vi "Run.vi"(8 "error in (no error)":errorcluster, 11 "LINX in":refnum<class "LINX.lvclass">) -> (0 "error out":errorcluster, 3 "LINX out":refnum<class "LINX.lvclass">)   [LabVIEW 2019, in "LINX.lvlib" / "LINX.lvclass"]
doc: "<b>Execution System:</b> Data Acquisition"
uses:
  LINX.lvclass
  <vilib>/MakerHub/LINX/Private/Local IO/LinxAnalogRead.vi
  <vilib>/MakerHub/LINX/Public/Utilities/Check Channel.vi
  <vilib>/MakerHub/LINX/Private/Local IO/LinxDigitalRead.vi
  <vilib>/MakerHub/LINX/Private/Utilties/Generate Error.vi
  Packed Libraries/Messaging.lvlibp/Send.vi
  <vilib>/MakerHub/LINX/Public/Peripherals/Analog/Analog Read N Chans.vi
  <vilib>/MakerHub/LINX/Public/Peripherals/Digital/Digital Read N Chans.vi
  <vilib>/MakerHub/LINX/Public/Utilities/Open Serial.vi
  Plugin Interfaces/Controller Interface/Controller Interface.lvlibp/Controller Interface Class/Controller Interface.lvclass
  <vilib>/MakerHub/LINX/LMH-LINX.lvlib
  C:/github/dataflowg/dataflow-dj/src/Plugin Interfaces/Controller Interface/Controller Interface.lvlibp/Controller Interface Class/Controller Interface.lvclass
panel:
  out "Error":errorcluster
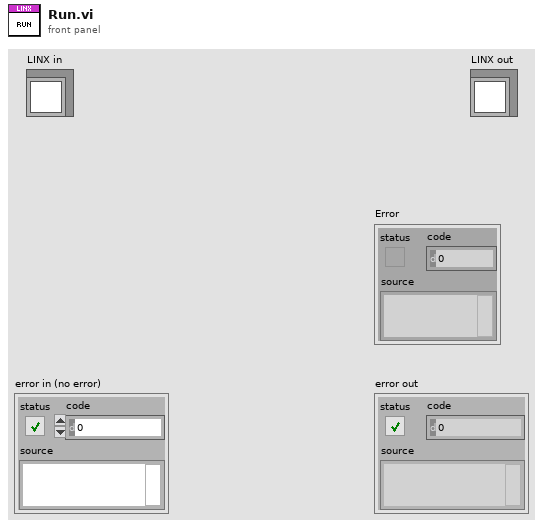
[diagram p1: front panel]
types:
  T1 = typedef "LINX.lvlib/LINX.lvclass/LINX Control Shortcut.ctl" = cluster{"Channel Type":T2, "Channel Number":u8, "Message Queue":string, "Event":string, "Target":string, "Momentary":bool, "Data":variant}
  T2 = typedef "LINX.lvlib/LINX.lvclass/LINX Channel Type.ctl" = enum16{"DI", "AI"}
  T3 = cluster{"value":string, "value":i32, T1[], T1[]}[]
  T4 = typedef "LMH-LINX.lvlib/LINX Ref.ctl" = cluster{"IO":T5, "Interface":T6, "LINX Device Config":T7}
  T5 = typedef "LMH-LINX.lvlib/Platform.ctl" = enum16{"Remote", "Local"}
  T6 = typedef "LMH-LINX.lvlib/Interface.ctl" = enum16{"Serial", "TCP"}
  T7 = typedef "LMH-LINX.lvlib/Device.lvlib/LINX Device Config.ctl" = cluster{"Interface":T6, "COM Port":refnum<visa-resource-name>, "TCP Configuration":T8, "Device Family":u8, "Device ID":u8, "Device Name":string, "TCP Ref":refnum<k5>, "Channels":T9}
  T8 = typedef "LMH-LINX.lvlib/Device.lvlib/TCP Config.ctl" = cluster{"IP Address":string, "Port":u16}
  T9 = typedef "LMH-LINX.lvlib/Channels.ctl" = cluster{"DI":u8[], "DO":u8[], "AI":u8[], "AO":u8[], "PWM":u8[], "QE":u8[], "UART":u8[], "I2C 2":u8[], "SPI":u8[], "CAN":u8[], "Servo":u8[], "AI Ref (V)":dbl, "AI Resolution (Bits)":u8, "AO Ref (V)":dbl, "AO Resolution (Bits)":u8}
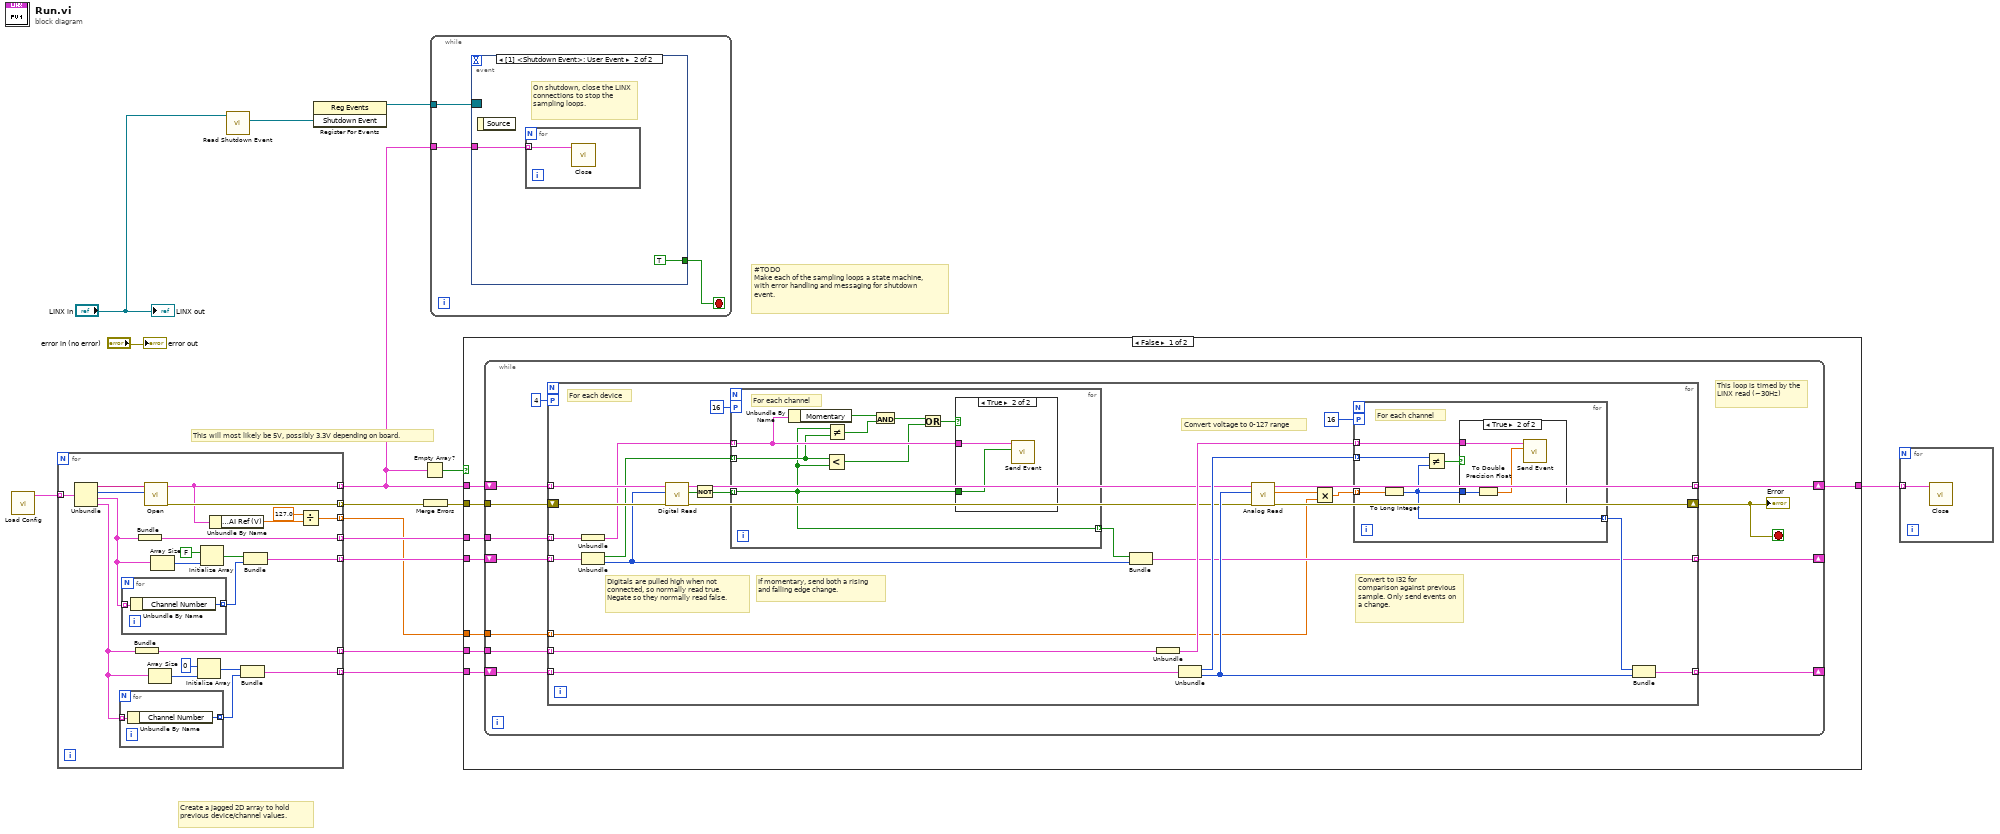
[diagram p0: block diagram]
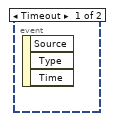
[diagram p5: hidden frame]
diagram:
  # "This will most likely be 5V, possibly 3.3V depending on board."
  # "#TODO\nMake each of the sampling loops a state machine, with error handling and messaging for shutdown event."
  # "Create a jagged 2D array to hold previous device/channel values."
  n1 = call "Load Config.vi"() -> ("Array"=w5:T3)  [unwired: 10 in, 1 out]
  n2 = for {
    tunnel: [w33] -> w15 mode=indexing
    tunnel: [w37] -> w14 mode=indexing
    tunnel: [w19] -> w10 mode=indexing
    tunnel: [w28] -> w12 mode=indexing
    tunnel: w5 -> [w31] mode=indexing
    tunnel: [w21] -> w4 mode=indexing
    tunnel: [w20] -> w3 mode=indexing
    tunnel: [w16] -> w1 mode=indexing
    n3 = Unbundle(w31) -> ("value"=w30:string, "value"=w29:i32, w23:T1[], w27:T1[])
    n4 = for {
      tunnel: w27 -> [w41] mode=indexing
      tunnel: [w40] -> w32 mode=indexing
      n5 = Unbundle By Name(w41) -> ("Channel Number"=w40:u8)
    }
    n6 = for {
      tunnel: w23 -> [w39] mode=indexing
      tunnel: [w38] -> w26 mode=indexing
      n7 = Unbundle By Name(w39) -> ("Channel Number"=w38:u8)
    }
    n8 = Bundle(w27) -> (w28:cluster{T1[]})  [unwired: 1 in]
    n9 = Bundle(w23) -> (w21:cluster{T1[]})  [unwired: 1 in]
    n10 = call-poly <vilib>:"Open.vi"("Baud Rate Override"=w29, "Serial Port"=w30) -> ("Error Out"=w33:errorcluster, "LINX Resource"=w19:T4)  [unwired: 7 in, 1 out]
    n11 = Array Size(array=w27) -> (size(s)=w35:i32)
    n12 = Array Size(array=w23) -> (size(s)=w24:i32)
    n13 = Initialize Array(0 ("element"), w35) -> (w34:i32[])
    n14 = Initialize Array(FALSE, w24) -> (w25:bool[])
    n15 = Unbundle By Name(w19) -> ("LINX Device Config.Channels.AI Ref (V)"=w18:dbl)
    n16 = Bundle(w34, w32) -> (w37:cluster{i32[], u8[]})  [unwired: 1 in]
    n17 = Bundle(w25, w26) -> (w20:cluster{bool[], u8[]})  [unwired: 1 in]
    n18 = Divide(x=127.0 ("y"), y=w18) -> (x/y=w16:dbl)
  }
  n19 = call "Read Shutdown Event.vi"("Controller Interface in"="LINX in") -> ("Shutdown Event"=w6:refnum<user-event>)  [unwired: 9 in, 1 out]
  n20 = register-events(w6) -> (reference out=w13:refnum<event-registration>)  [unwired: 2 in, 1 out]
  n21 = Empty Array?(array=w10) -> (empty?=w9:bool)
  n22 = Merge Errors(w15) -> (w11:errorcluster)
  n23 = while {
    tunnel: w13 -> [w44]
    tunnel: w10 -> [w42]
    stop <- w43 stop-if-true
    n24 = event shown="[1] <Shutdown Event>: User Event" {
      selector: w44 -> [_ _]
      dyn-events: _ -> [_ _]
      timeout: _ -> [_ _]
      tunnel: [_ TRUE] -> w43
      tunnel: w42 -> [_ w45]
      event Timeout {
        n25 = event-data() -> ()  [unwired: 1 in, 3 out]
      }
      event User Event {
        # "On shutdown, close the LINX connections to stop the sampling loops."
        n26 = event-data() -> ()  [unwired: 1 in, 1 out]
        n27 = for {
          tunnel: w45 -> [w47] mode=indexing
          n28 = call <vilib>:"Close.vi"("LINX Resource"=w47) -> ()  [unwired: 10 in, 1 out]
        }
      }
    }
  }
  n29 = case shown="False" w9 {
    tunnel: w14 -> [w55 _]
    tunnel: w12 -> [w54 _]
    tunnel: w11 -> [w53 _]
    tunnel: w10 -> [w52 w113]
    tunnel: w4 -> [w51 _]
    tunnel: w3 -> [w50 _]
    tunnel: [w49 w113] -> w2
    tunnel: w1 -> [w48 _]
    frame False {
      n30 = while {
        tunnel: w53 -> [w66]
        tunnel: w54 -> [w64]
        shift-right: [w63] -> _
        shift-left: w55 -> [w65]
        shift-right: [w62] -> w49
        shift-left: w52 -> [w67]
        tunnel: w51 -> [w60]
        shift-right: [w58] -> _
        shift-left: w50 -> [w59]
        tunnel: w48 -> [w56]
        stop <- w61 stop-if-true
        # "This loop is timed by the LINX read (~30Hz)"
        n31 = for {
          tunnel: w67 -> [w82] mode=indexing
          tunnel: w65 -> [w91] mode=indexing
          tunnel: w64 -> [w94] mode=indexing
          tunnel: [w89] -> w63 mode=indexing
          shift-right: [w88] -> w61
          shift-left: w66 -> [w81]
          tunnel: [w87] -> w62 mode=indexing
          tunnel: w60 -> [w85] mode=indexing
          tunnel: w59 -> [w84] mode=indexing
          tunnel: [w74] -> w58 mode=indexing
          workers-P: 4 -> [_]
          tunnel: w56 -> [w70] mode=indexing
          # "Convert voltage to 0-127 range"
          # "Digitals are pulled high when not connected, so normally read true. Negate so they normally read false."
          # "Convert to I32 for comparison against previous sample. Only send events on a change."
          # "If momentary, send both a rising and falling edge change."
          # "For each device"
          n32 = Unbundle(w85) -> (w78:T1[])
          n33 = Unbundle(w84) -> (w77:bool[], w76:u8[])
          n34 = call-poly <vilib>:"Digital Read.vi"("Error In"=w81, "DI Channels"=w76, "LINX Resource"=w82) -> ("Error Out"=w80:errorcluster, "Values"=w79:bool[], "LINX Resource"=w83:T4)  [unwired: 6 in]
          n35 = Not(x=w79) -> (.not. x?=w73:bool[])
          n36 = for {
            tunnel: w73 -> [w97] mode=indexing
            tunnel: w78 -> [w101] mode=indexing
            tunnel: w77 -> [w98] mode=indexing
            tunnel: [w97] -> w75 mode=indexing
            workers-P: 16 -> [_]
            # "For each channel"
            n37 = Unbundle By Name(w101) -> ("Momentary"=w100:bool)
            n38 = Less?(x=w98, y=w97) -> (x < y?=w96:bool)
            n39 = Not Equal?(x=w97, y=w98) -> (x != y?=w102:bool)
            n40 = And(x=w100, y=w102) -> (x .and. y?=w99:bool)
            n41 = Or(x=w99, y=w96) -> (x .or. y?=w95:bool)
            n42 = case shown="True" w95 {
              tunnel: w101 -> [_ w104]
              tunnel: w97 -> [_ w103]
              frame False {
              }
              frame True {
                n43 = call "Send Event.vi"("Data"=w103, "LINX Shortcut"=w104) -> ()  [unwired: 10 in]
              }
            }
          }
          n44 = Bundle(w75, w76) -> (w74:cluster{bool[], u8[]})  [unwired: 1 in]
          n45 = Unbundle(w94) -> (w90:T1[])
          n46 = Unbundle(w91) -> (w92:i32[], w86:u8[])
          n47 = call-poly <vilib>:"Analog Read.vi"("Error In"=w80, "AI Channel(s)"=w86, "LINX Resource"=w83) -> ("Error Out"=w88:errorcluster, "Voltages"=w69:dbl[], "LINX Resource"=w87:T4)  [unwired: 5 in, 1 out]
          n48 = Multiply(x=w69, y=w70) -> (x*y=w68:dbl[])
          n49 = for {
            tunnel: w68 -> [w105] mode=indexing
            tunnel: w92 -> [w109] mode=indexing
            tunnel: w90 -> [w108] mode=indexing
            tunnel: [w106] -> w93 mode=indexing
            workers-P: 16 -> [_]
            # "For each channel"
            n50 = To Long Integer(number=w105) -> (32bit integer=w106:i32)
            n51 = Not Equal?(x=w109, y=w106) -> (x != y?=w107:bool)
            n52 = case shown="True" w107 {
              tunnel: w108 -> [_ w111]
              tunnel: w106 -> [_ w112]
              frame False {
              }
              frame True {
                n53 = To Double Precision Float(number=w112) -> (double precision float=w110:dbl)
                n54 = call "Send Event.vi"("Data"=w110, "LINX Shortcut"=w111) -> ()  [unwired: 10 in]
              }
            }
          }
          n55 = Bundle(w93, w86) -> (w89:cluster{i32[], u8[]})  [unwired: 1 in]
        }
        "Error" <- w61
      }
    }
    frame True {
    }
  }
  n56 = for {
    tunnel: w2 -> [w114] mode=indexing
    n57 = call <vilib>:"Close.vi"("LINX Resource"=w114) -> ()  [unwired: 10 in, 1 out]
  }
  "error out" <- "error in (no error)"
  "LINX out" <- "LINX in"
